vi "Migrate.vi"(8 "error in (no error)":errorcluster, 10 "Migration File Path":path, 11 "SQLite Connection in":refnum<class "Connection.lvclass">) -> (0 "error out":errorcluster, 3 "SQLite Connection out":refnum<class "Connection.lvclass">)   [LabVIEW 2024, in "DBMigrations.lvlib"]
doc: "Apply migration (.sql file) to database."
uses:
  DBMigrations.lvlib
  <vilib>/drjdpowell/SQLite Library/SQL Connection/Connection.lvclass
  <vilib>/Utility/error.llb/Trim Whitespace One-Sided.vi
  <vilib>/drjdpowell/SQLite Library/SQL Connection/Execute SQL (No results).vi
  <vilib>/drjdpowell/SQLite Library/SQLite.lvlib
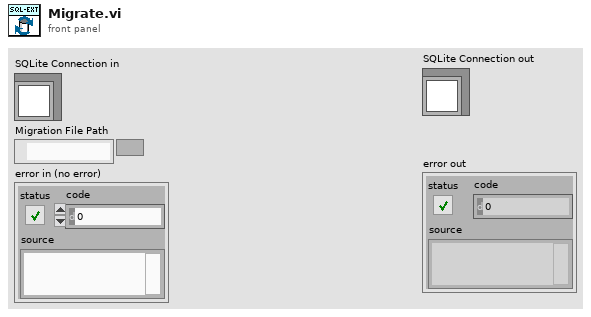
[diagram p1: front panel]
types:
  T1 = enum16{"open", "replace", "create", "open or create", "replace or create", "replace or create with confirmation"}
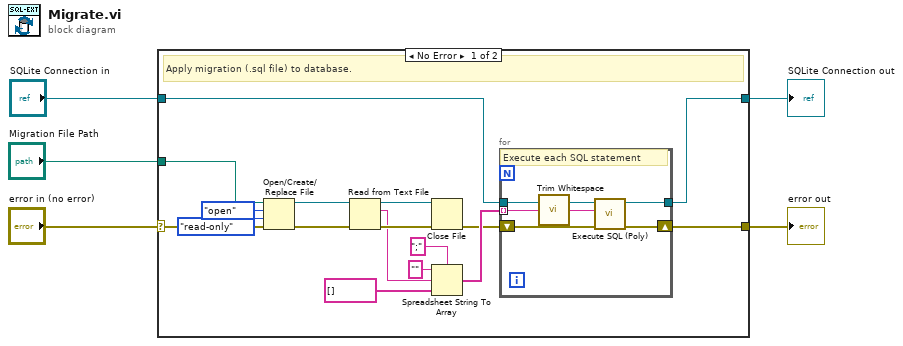
[diagram p0: block diagram]
diagram:
  n1 = case shown="No Error" "error in (no error)" {
    selector: "error in (no error)" -> [w6 w29]
    tunnel: "Migration File Path" -> [w12 _]
    tunnel: "SQLite Connection in" -> [w11 w30]
    tunnel: [w10 w30] -> w3
    tunnel: [w9 w29] -> w2
    frame No Error {
      # "Apply migration (.sql file) to database."
      n2 = Open/Create/Replace File(file path (use dialog)=w12, error in=w6, operation (0:open)=T1."open", access (0:read/write)=enum16{"read/write", "read-only", "write-only"}."read-only") -> (refnum out=w22:refnum<file>, error out=w20:errorcluster)  [unwired: 2 in, 1 out]
      n3 = Read from Text File(file (use dialog)=w22, error in=w20) -> (refnum out=w21:refnum<file>, text=w8:string, error out=w19:errorcluster)  [unwired: 2 in, 1 out]
      n4 = Close File(refnum=w21, error in=w19) -> (error out=w13:errorcluster)  [unwired: 1 out]
      n5 = Spreadsheet String To Array(delimiter (Tab)=";", format string="", spreadsheet string=w8, array type (2D Dbl)=string[] []) -> (array=w14:string[])
      n6 = for {
        tunnel: w14 -> [w28] mode=indexing
        shift-right: [w25] -> w9
        shift-left: w13 -> [w26]
        tunnel: w11 -> [w24]
        tunnel: [w23] -> w10
        # "Execute each SQL statement"
        n7 = call <vilib>:"Trim Whitespace.vi"("string"=w28) -> ("trimmed string"=w27:string)  [unwired: 1 in]
        n8 = call-poly <vilib>:"Execute SQL (Poly).vi"("error in (no error)"=w26, "SQL"=w27, "SQLite Connection in"=w24) -> ("error out"=w25:errorcluster, "SQLite Connection"=w23:refnum<class "Connection.lvclass">)  [unwired: 7 in]
      }
    }
    frame Error {
    }
  }
  "SQLite Connection out" <- w3
  "error out" <- w2
